vi "Stream State.vi"(8 "error in":errorcluster, 10 "set?":bool, 11 "state in":string) -> (0 "error out":errorcluster, 3 "state out":string)   [LabVIEW 2020, in "MCP Server.lvlib"]
doc: "Functional global that keeps the progress state of the streamed tools/call that is running: a JSON object {\"key\",\"last\",\"cancelled\",\"probe\"} written by Report Progress.vi and Cancel Requested.vi. \"key\" identifies the stream (the stream object of the request context), so a value left over from an earlier request is recognised and ignored.\n\nOne slot is enough because Handle MCP Request.vi runs one request at a time.\n\nset? TRUE stores state in; FALSE only reads. state out is the stored value after the call."
uses:
  MCP Server.lvlib
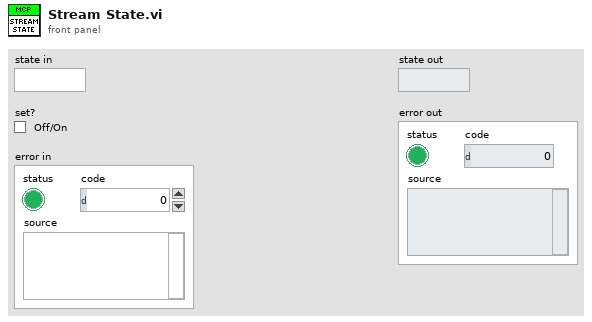
[diagram p1: front panel]
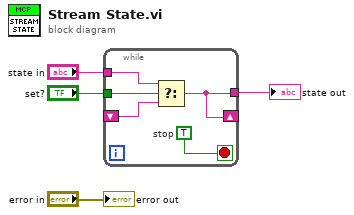
[diagram p0: block diagram]
diagram:
  n1 = while {
    tunnel: "state in" -> [w9]
    tunnel: "set?" -> [w8]
    shift-right: [w5] -> _
    shift-left: _ -> [w7]
    tunnel: [w5] -> w2
    stop <- w6 stop-if-true
    w6 = TRUE  # stop
    n2 = Select(t=w9, s=w8, f=w7) -> (s? t:f=w5:string)
  }
  "state out" <- w2
  "error out" <- "error in"
